vi "Test_Full_Run.vi"(8 "error in":errorcluster, 10 "Wait ms":i32=30000, 11 "Sequence Path":path=path "C:/Users/DynaAdmin/PycharmProjects/Universal-sequence-executor-AF/configs/sequences/vtu_actual_sequence.json") -> (0 "error out":errorcluster)   [LabVIEW 2026]
doc: "Full end-to-end run: Load -> Start -> wait (default 30 s, enough for all 5 steps) -> Normal Stop -> notify. The evidence is results/VTU_ACTUAL_SEQUENCE_001_*.csv written by Finish Sequence."
uses:
  src/Executor/Sequence Executor.lvclass
  <vilib>/ActorFramework/Message Enqueuer/Message Enqueuer.lvclass/Message Enqueuer.ctl
  src/Executor Messages/Load Sequence Msg/Load Sequence Msg.lvclass/Load Sequence Msg.ctl
  <vilib>/ActorFramework/Message Enqueuer/Enqueue.vi
  <vilib>/ActorFramework/Stop Msg/Stop Msg.lvclass
  src/Executor Messages/Load Sequence Msg/Load Sequence Msg.lvclass
  src/Executor Messages/Start Sequence Msg/Start Sequence Msg.lvclass
  <vilib>/ActorFramework/Message Priority Queue/Priority Enqueue.vi
  <vilib>/ActorFramework/Actor/Actor.lvclass
panel:
  out "Start error":errorcluster
  out "Load error":errorcluster
  out "Stopped cleanly":bool
  out "Feedback Chart":dbl
  out "Verdict":string
  out "Channel Values":string[][](array[string])
  out "Step Table":string[][](array[string])
  out "Step Index":i32
  out "Status":string
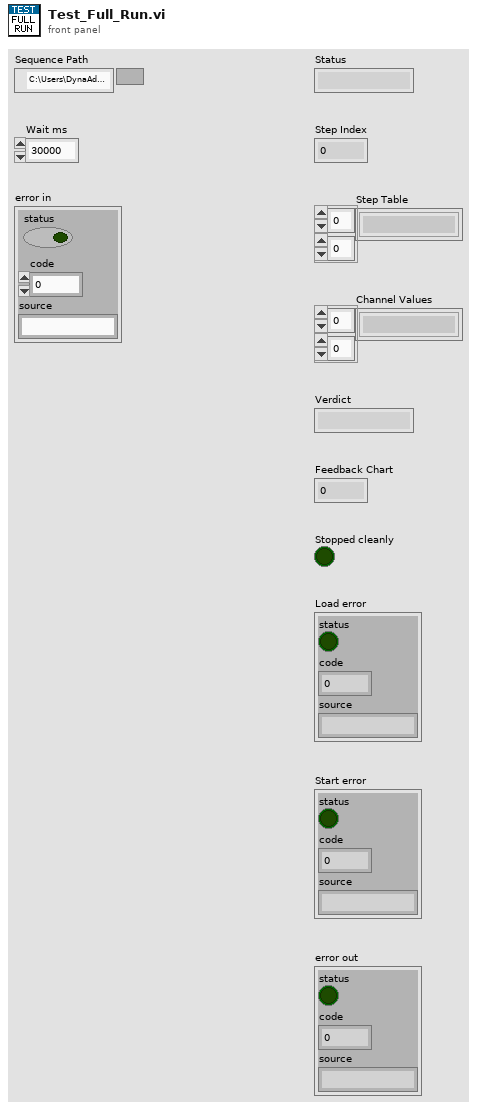
[diagram p1: front panel]
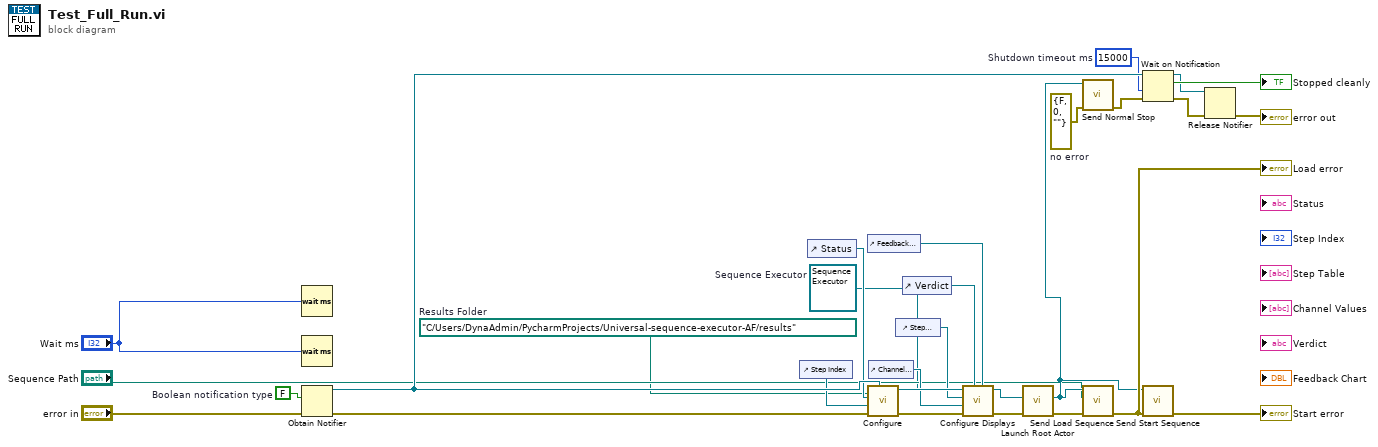
[diagram p0: block diagram]
diagram:
  w5 = path "C:/Users/DynaAdmin/PycharmProjects/Universal-sequence-executor-AF/results"  # Results Folder
  w4 = 15000  # Shutdown timeout ms
  w3 = errorcluster {"status"=FALSE, "code"=0, "source"=""}  # no error
  w2 = FALSE  # Boolean notification type
  w1 = refnum<class "Sequence Executor.lvclass"> refnum  # Sequence Executor
  n1 = Wait (ms)(milliseconds to wait="Wait ms") -> ()  [unwired: 1 out]
  n2 = Wait (ms)(milliseconds to wait="Wait ms") -> ()  [unwired: 1 out]
  n3 = Obtain Notifier(notification data type=w2, error in (no error)="error in") -> (notifier out=w15:refnum<notifier>, error out=w16:errorcluster)  [unwired: 2 in, 1 out]
  n4 = control-ref of="Step Index"() -> (w10:refnum<vi>)
  n5 = control-ref of="Status"() -> (w9:refnum<vi>)
  n6 = control-ref of="Feedback Chart"() -> (w14:refnum<vi>)
  n7 = call "Configure.vi"("Results Folder"=w5, "Stopped Notification"=w15, "error in"=w16, "Step Index Display"=w10, "Status Display"=w9, "Sequence Executor in"=w1) -> ("error out"=w18:errorcluster, "Sequence Executor out"=w17:refnum<class "Sequence Executor.lvclass">)  [unwired: 4 in]
  n8 = control-ref of="Channel Values"() -> (w12:refnum<vi>)
  n9 = control-ref of="Step Table"() -> (w11:refnum<vi>)
  n10 = control-ref of="Verdict"() -> (w13:refnum<vi>)
  n11 = call "Configure Displays.vi"("Feedback Chart"=w14, "Verdict Display"=w13, "error in"=w18, "Channel Values Display"=w12, "Step Table Display"=w11, "Sequence Executor in"=w17) -> ("error out"=w20:errorcluster, "Sequence Executor out"=w19:refnum<class "Sequence Executor.lvclass">)  [unwired: 4 in]
  n12 = call <vilib>:"Launch Root Actor.vi"("error in (no error)"=w20, "Actor"=w19) -> ("error out"=w22:errorcluster, "Actor's Enqueuer"=w21:refnum<class "Message Enqueuer.lvclass">)  [unwired: 8 in]
  n13 = call <vilib>:"Send Normal Stop.vi"("error in (no error)"=w3, "Message Enqueuer"=w21) -> ("error out"=w25:errorcluster)  [unwired: 9 in]
  n14 = call "Send Load Sequence.vi"("error in (no error)"=w22, "path"="Sequence Path", "Message Enqueuer"=w21) -> ("error out"=w23:errorcluster)  [unwired: 7 in, 1 out]
  "Load error" <- w23
  n15 = Wait on Notification(notifier=w15, timeout in ms (-1)=w4, error in (no error)=w25) -> (notifier out=w26:refnum<notifier>, notification=→"Stopped cleanly":bool, error out=w28:errorcluster)  [unwired: 1 in, 1 out]
  n16 = call "Send Start Sequence.vi"("error in (no error)"=w23, "Message Enqueuer"=w21) -> ("error out"=→"Start error":errorcluster)  [unwired: 8 in, 1 out]
  n17 = Release Notifier(notifier=w26, error in (no error)=w28) -> (error out=→"error out":errorcluster)  [unwired: 1 in, 2 out]
